vi "OwnCompat20261012_Native_GetForInfo.vi"() -> ()   [LabVIEW 2024]
panel:
  out "error out":errorcluster caption="错误输出"
  out "diagram_id":u32
  in  "diagram_id type":u32
  in  "for_id":u32
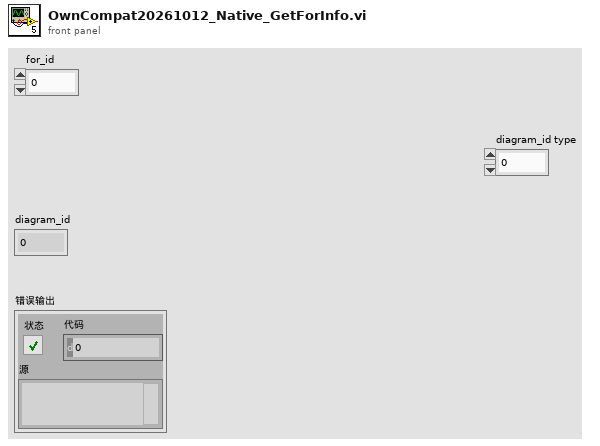
[diagram p1: front panel]
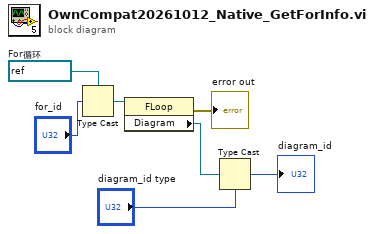
[diagram p0: block diagram]
diagram:
  w6 = refnum<vi> refnum  # For循环
  n1 = Type Cast ("强制类型转换")(type=w6, x="for_id") -> (*(type *) &x=w5:refnum<vi>)
  n2 = property on="属性节点" class="FLoop"(reference=w5) -> (error out=→"error out":errorcluster, "Diagram"=w4:refnum<vi>)  [unwired: 1 in, 1 out]
  n3 = Type Cast ("强制类型转换")(type="diagram_id type", x=w4) -> (*(type *) &x=→"diagram_id":u32)
